vi "Reset_Fault.vi"(8 "error in (no error)":errorcluster, 11 "Motor in":refnum<class "Motor.lvclass">) -> (0 "error out":errorcluster, 3 "Motor out":refnum<class "Motor.lvclass">)   [LabVIEW 2021, in "Motor.lvclass"]
uses:
  Motor.lvclass
  Motor.lvclass/Motor.ctl
  ServoDrive/ServoDrive.lvclass
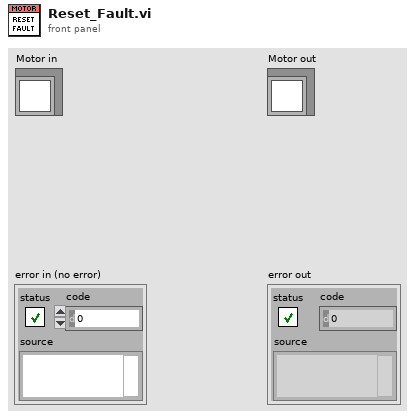
[diagram p1: front panel]
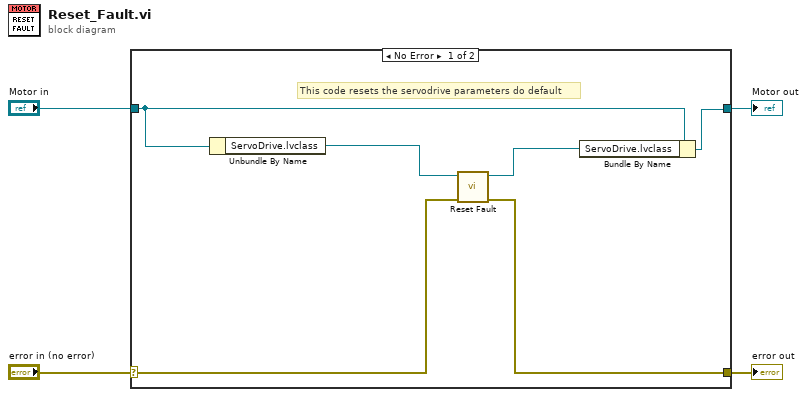
[diagram p0: block diagram]
diagram:
  n1 = case shown="No Error" "error in (no error)" {
    selector: "error in (no error)" -> [w7 w12]
    tunnel: [w6 w12] -> w3
    tunnel: [w9 w11] -> w1
    tunnel: "Motor in" -> [w10 w11]
    frame No Error {
      # "This code resets the servodrive parameters do default"
      n2 = Unbundle By Name(w10) -> ("ServoDrive.lvclass"=w8:refnum<class "ServoDrive.lvclass">)
      n3 = call-dynamic "Reset Fault.vi"("error in (no error)"=w7, "ServoDrive in"=w8) -> ("error out"=w6:errorcluster, "ServoDrive out"=w5:refnum<class "ServoDrive.lvclass">)  [unwired: 8 in]
      n4 = Bundle By Name(cluster=w10, "ServoDrive.lvclass"=w5) -> (w9:refnum<class "Motor.lvclass">)
    }
    frame Error {
    }
  }
  "error out" <- w3
  "Motor out" <- w1
